vi "constant-1-normal.vi"() -> ()   [LabVIEW 2026]
panel:
  out "Numeric":i32
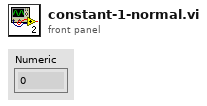
[diagram p1: front panel]
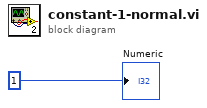
[diagram p0: block diagram]
diagram:
  "Numeric" <- 1
